vi "Draw Circle(SubVI).vi"(11 "Circles":T2(array[cluster])) -> (0 "element":T1, 2 "Score":dbl, 3 "Bounding Rectangle out":T3)   [LabVIEW 2014]
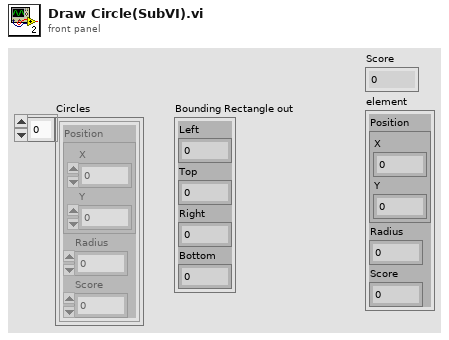
[diagram p1: front panel]
types:
  T1 = cluster{"Position":cluster{"X":sgl, "Y":sgl}, "Radius":dbl, "Score":dbl}
  T2 = cluster{"Position":cluster{"X":sgl, "Y":sgl}, "Radius":dbl, "Score":dbl}[]
  T3 = cluster{"Left":i32, "Top":i32, "Right":i32, "Bottom":i32}
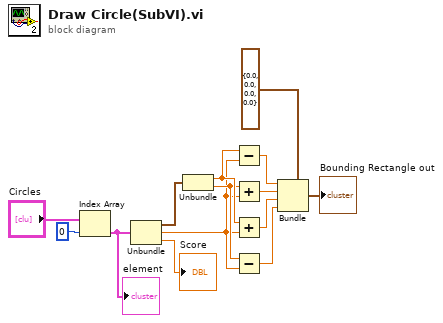
[diagram p0: block diagram]
diagram:
  n1 = Index Array(array="Circles", index=0) -> (element=w1:T1)
  "element" <- w1
  n2 = Unbundle(w1) -> ("Position"=w12:cluster{"X":sgl, "Y":sgl}, "Radius"=w8:dbl, "Score"=→"Score":dbl)
  n3 = Unbundle(w12) -> ("X"=w10:sgl, "Y"=w9:sgl)
  n4 = Subtract(x=w10, y=w8) -> (x-y=w7:dbl)
  n5 = Add(x=w9, y=w8) -> (x+y=w6:dbl)
  n6 = Add(x=w10, y=w8) -> (x+y=w5:dbl)
  n7 = Subtract(x=w9, y=w8) -> (x-y=w4:dbl)
  n8 = Bundle(cluster=cluster{dbl, dbl, dbl, dbl} {0.0, 0.0, 0.0, 0.0}, w7, w6, w5, w4) -> (→"Bounding Rectangle out":cluster{dbl, dbl, dbl, dbl})
